vi "Waveform and Laser Controls V7.vi"() -> ()   [LabVIEW 2014]
uses:
  Waveform Scan Parameters.ctl
  <vilib>/Platform/TimedLoop/XDataNode/timing_clust.ctl
  <vilib>/Platform/TimedLoop/XDataNode/nitl_modes.ctl
  <vilib>/Platform/TimedLoop/XDataNode/wakeup.ctl
  <vilib>/rvi/Emulation/niFpgaGetClockAttributes.vi
  <vilib>/rvi/Emulation/niFpgaSctlEmulationGetInTimedLoop.vi
  <vilib>/rvi/Emulation/niFpgaEmulationReportErrorSimple.vi
  <vilib>/rvi/Emulation/niFpgaProcessEmulError.vi
  <vilib>/rvi/eio/common/nirviEmuTemplateMethod_errors.vi
  <vilib>/rvi/Emulation/niFpgaCriticalErrorInLSC.vi
  <vilib>/rvi/Memory/Memory_Emulation/nirvimemoryFastEmulation.vi
  <vilib>/rvi/Memory/Memory_Emulation/nirvimemoryEmulation.vi
  <vilib>/rvi/Emulation/niFpgaEmulationIsFPGAContextNoSignature.vi
  <vilib>/rvi/DataTransferAndStorage/Container/Common/niFpgaContainerGetUniqueNameForEmu.vi
  <vilib>/rvi/errors/nirviReportUnexpectedCaseInternalError (U32).vi
  <vilib>/rvi/Memory/Memory_Emulation/niFpgaMemoryEmulationCacheClearOnFirstRun.vi
  <vilib>/rvi/Memory/Memory_Emulation/nirvimemoryEmulationManagerCache_MakeExclusive.vi
  <vilib>/rvi/Memory/Memory_Emulation/niFpgaMemoryEmulationValidateCache.vi
  <vilib>/rvi/Memory/Memory_Emulation/nirvimemoryEmulationManagerCache_InsertValue.vi
  <vilib>/Utility/error.llb/Clear Errors.vi
  <vilib>/rvi/Memory/Memory_Emulation/nirvimemoryEmulationManagerCache_ReleaseExclusive.vi
  <vilib>/rvi/Memory/Memory_Emulation/nirvimemoryEmulationManagerCache_GetValue.vi
  <vilib>/rvi/Memory/Memory_Emulation/nirvimemoryEmulationManagerCache_SetValue.vi
  <vilib>/eio/EIONode/EIONode.xnode
  <vilib>/rvi/DataTransferAndStorage/Container/XNode/niFpgaContainer.xnode
  <vilib>/Platform/TimedLoop/XDataNode/XDataNode.xnode
  <vilib>/rvi/DataTransferAndStorage/Register/Emulation/niFpgaRegisterEmulation.vi
  <vilib>/Platform/TimedLoop/XDataNode/XDNodeRunTimeDep.lvlib
panel:
  out "frame counter":u16
  in  "Current Frame":u16
  in  "Lower Shutter Command":bool
  in  "Upper Shutter Command":bool
  out "Lower Shutter Status":bool
  out "Upper Shutter Status":bool
  in  "stop":bool
  in  "775 AOM (I16)":i16=16500
  out "Laser Blank Trigger":bool
  in  "Laser On Time (Ticks)":u8=8
  in  "Sequences":u8=4
  in  "Laser Delay (Ticks)":u8
  in  "Laser States":u32
  in  "Blanking Off/Manual":bool
  in  "Z Piezo Axis":i16
  in  "Y Piezo Axis":i16
  in  "X Piezo Axis":i16
  out "End Linear Ramp":bool
  in  "End of Linear Ramp":u32
  in  "Z Stack Start Position (I16)":i16
  in  "Frames Per Z Step":u16
  in  "Number of Z Steps":u16
  in  "Z Step Size (I16)":i16
  in  "Stop Sync Signal":bool
  in  "Accums Per Line":u32[](array[numeric])=[0, 0, 0, 0]
  in  "Number of Lines":u32
  out "Frame Trigger":bool
  in  "Reset Position Error":bool
  in  "Galvo 1 Position (I16)":i16
  in  "Galvo 2 Position (I16)":i16
  in  "WF 3 Data Loaded":bool
  in  "WF 2 Data Loaded":bool
  in  "Waveform Scan Parameters":T1={"Scanning Mode"=0, "Fast Axis WF Length (Elements)"=0, "Fast Axis Sample Period (Ticks)"=40, "Slow Axis 1 WF Length (Elements)"=0, "Slow Axis 1 Sample Period (Ticks)"=40, "Slow Axis 1 Delay (25 ns) Steps"=40, "Slow Axis 2 WFLength (Elements)"=0, "Slow Axis 2 Sample Period (Ticks)"=40, "Slow Axis 2 Delay (25 ns) Steps"=40}
  in  "Resonant Mirror":T2
  in  "Galvo Mirror 2":T3
  in  "Galvo Mirror 1":T3
  in  "Start Waveforms":bool
  in  "Unused Axis Offset":i16
  in  "Slow Axis 2 Waveform Element":i16
  in  "Fast Axis Waveform Element":i16
  in  "Slow Axis 1 Waveform Element":i16
  in  "WF 1 Data Loaded":bool
  # "V2 - Adding in a line clock\nV3 - Cluster Scan Parameters"
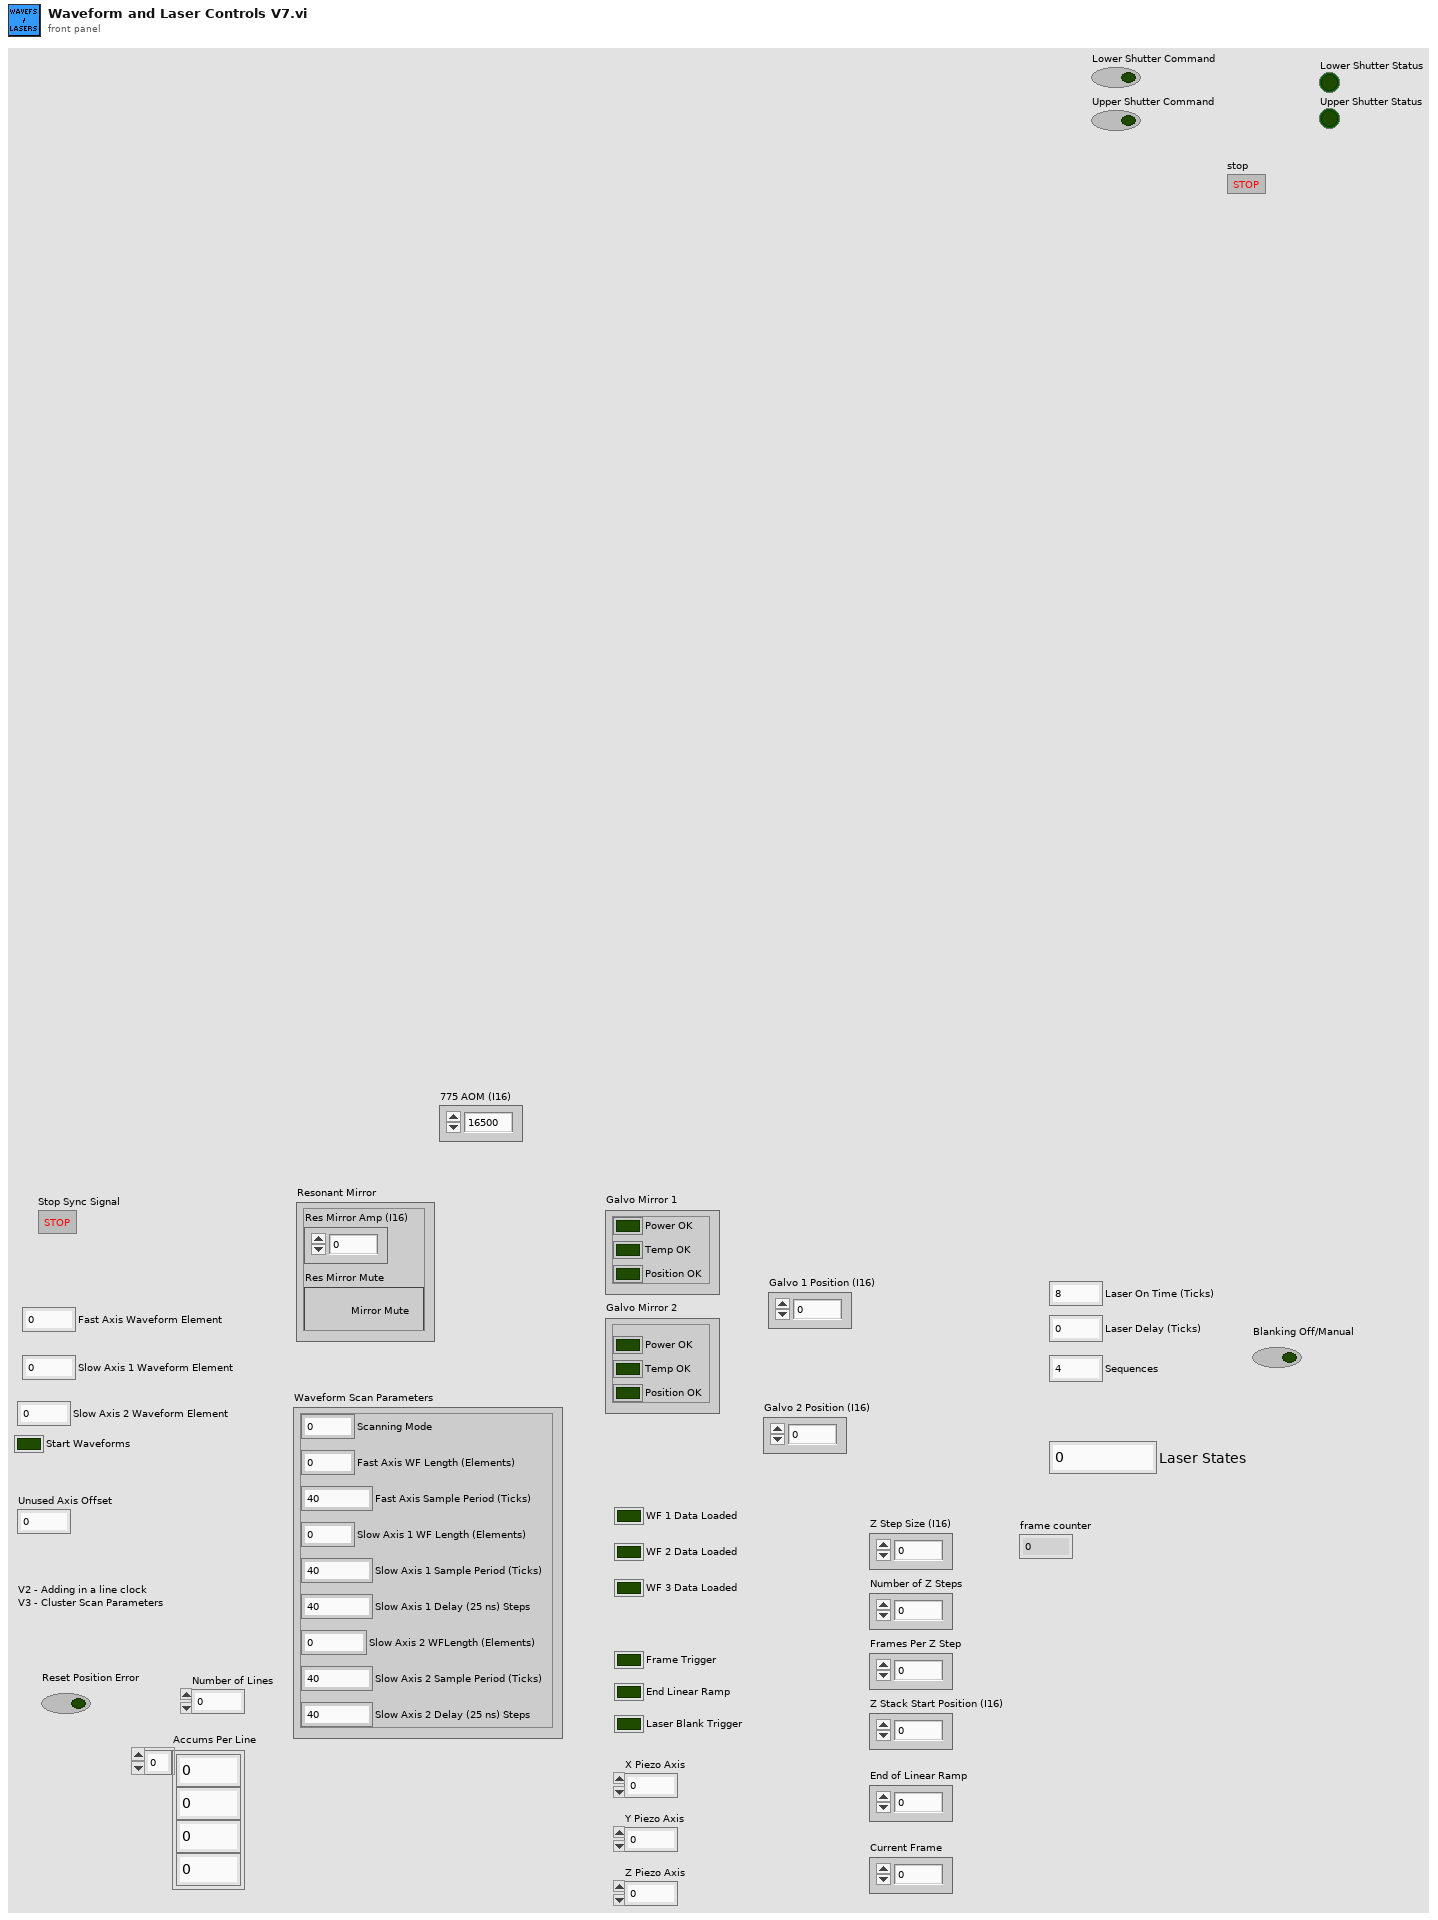
[diagram p1: front panel]
types:
  T1 = typedef "Waveform Scan Parameters.ctl" = cluster{"Scanning Mode":u8, "Fast Axis WF Length (Elements)":i32, "Fast Axis Sample Period (Ticks)":u32, "Slow Axis 1 WF Length (Elements)":i32, "Slow Axis 1 Sample Period (Ticks)":u32, "Slow Axis 1 Delay (25 ns) Steps":i32, "Slow Axis 2 WFLength (Elements)":i32, "Slow Axis 2 Sample Period (Ticks)":u32, "Slow Axis 2 Delay (25 ns) Steps":i32}
  T2 = cluster{"Res Mirror Amp (I16)":i16, "Res Mirror Mute":bool}
  T3 = cluster{"Power OK":bool, "Temp OK":bool, "Position OK":bool}
  T4 = typedef "XDNodeRunTimeDep.lvlib/timing_clust.ctl" = cluster{"Expected End [f-1]":u64, "Actual End [f-1]":u64, "Finished Late? [f-1]":bool, "Expected End [i-1]":u64, "Actual End [i-1]":u64, "Finished Late? [i-1]":bool, "Expected Start [i]":u64, "Actual Start [i]":u64, "Expected Start [f]":u64, "Actual Start [f]":u64, "Source Name":string, "Structure Name":string, "Period":i64, "Deadline":i64, "Offset":i64, "Start":i64, "Priority":i32, "Timeout":i32, "Mode":T5, "Wakeup Reason":T6, "Error":errorcluster, "Source Type":string, "Secondary Source Type":string, "Global End Time":u64, "Global Start Time":u64, "Frame Duration":u64, "Iteration Duration":u64, "Assigned CPU":i32, "I/O Scan Engine Mode":u32}
  T5 = typedef "XDNodeRunTimeDep.lvlib/nitl_modes.ctl" = enum32{"No Change", "Process missed periods, maintain original phase", "Discard missed periods, maintain original phase", "Process missed periods, ignore original phase", "Discard missed periods, ignore original phase"}
  T6 = typedef "XDNodeRunTimeDep.lvlib/wakeup.ctl" = enum32{"Normal", "Aborted", "Asynchronous wakeup", "Timing source error", "Timed loop error", "Timeout"}
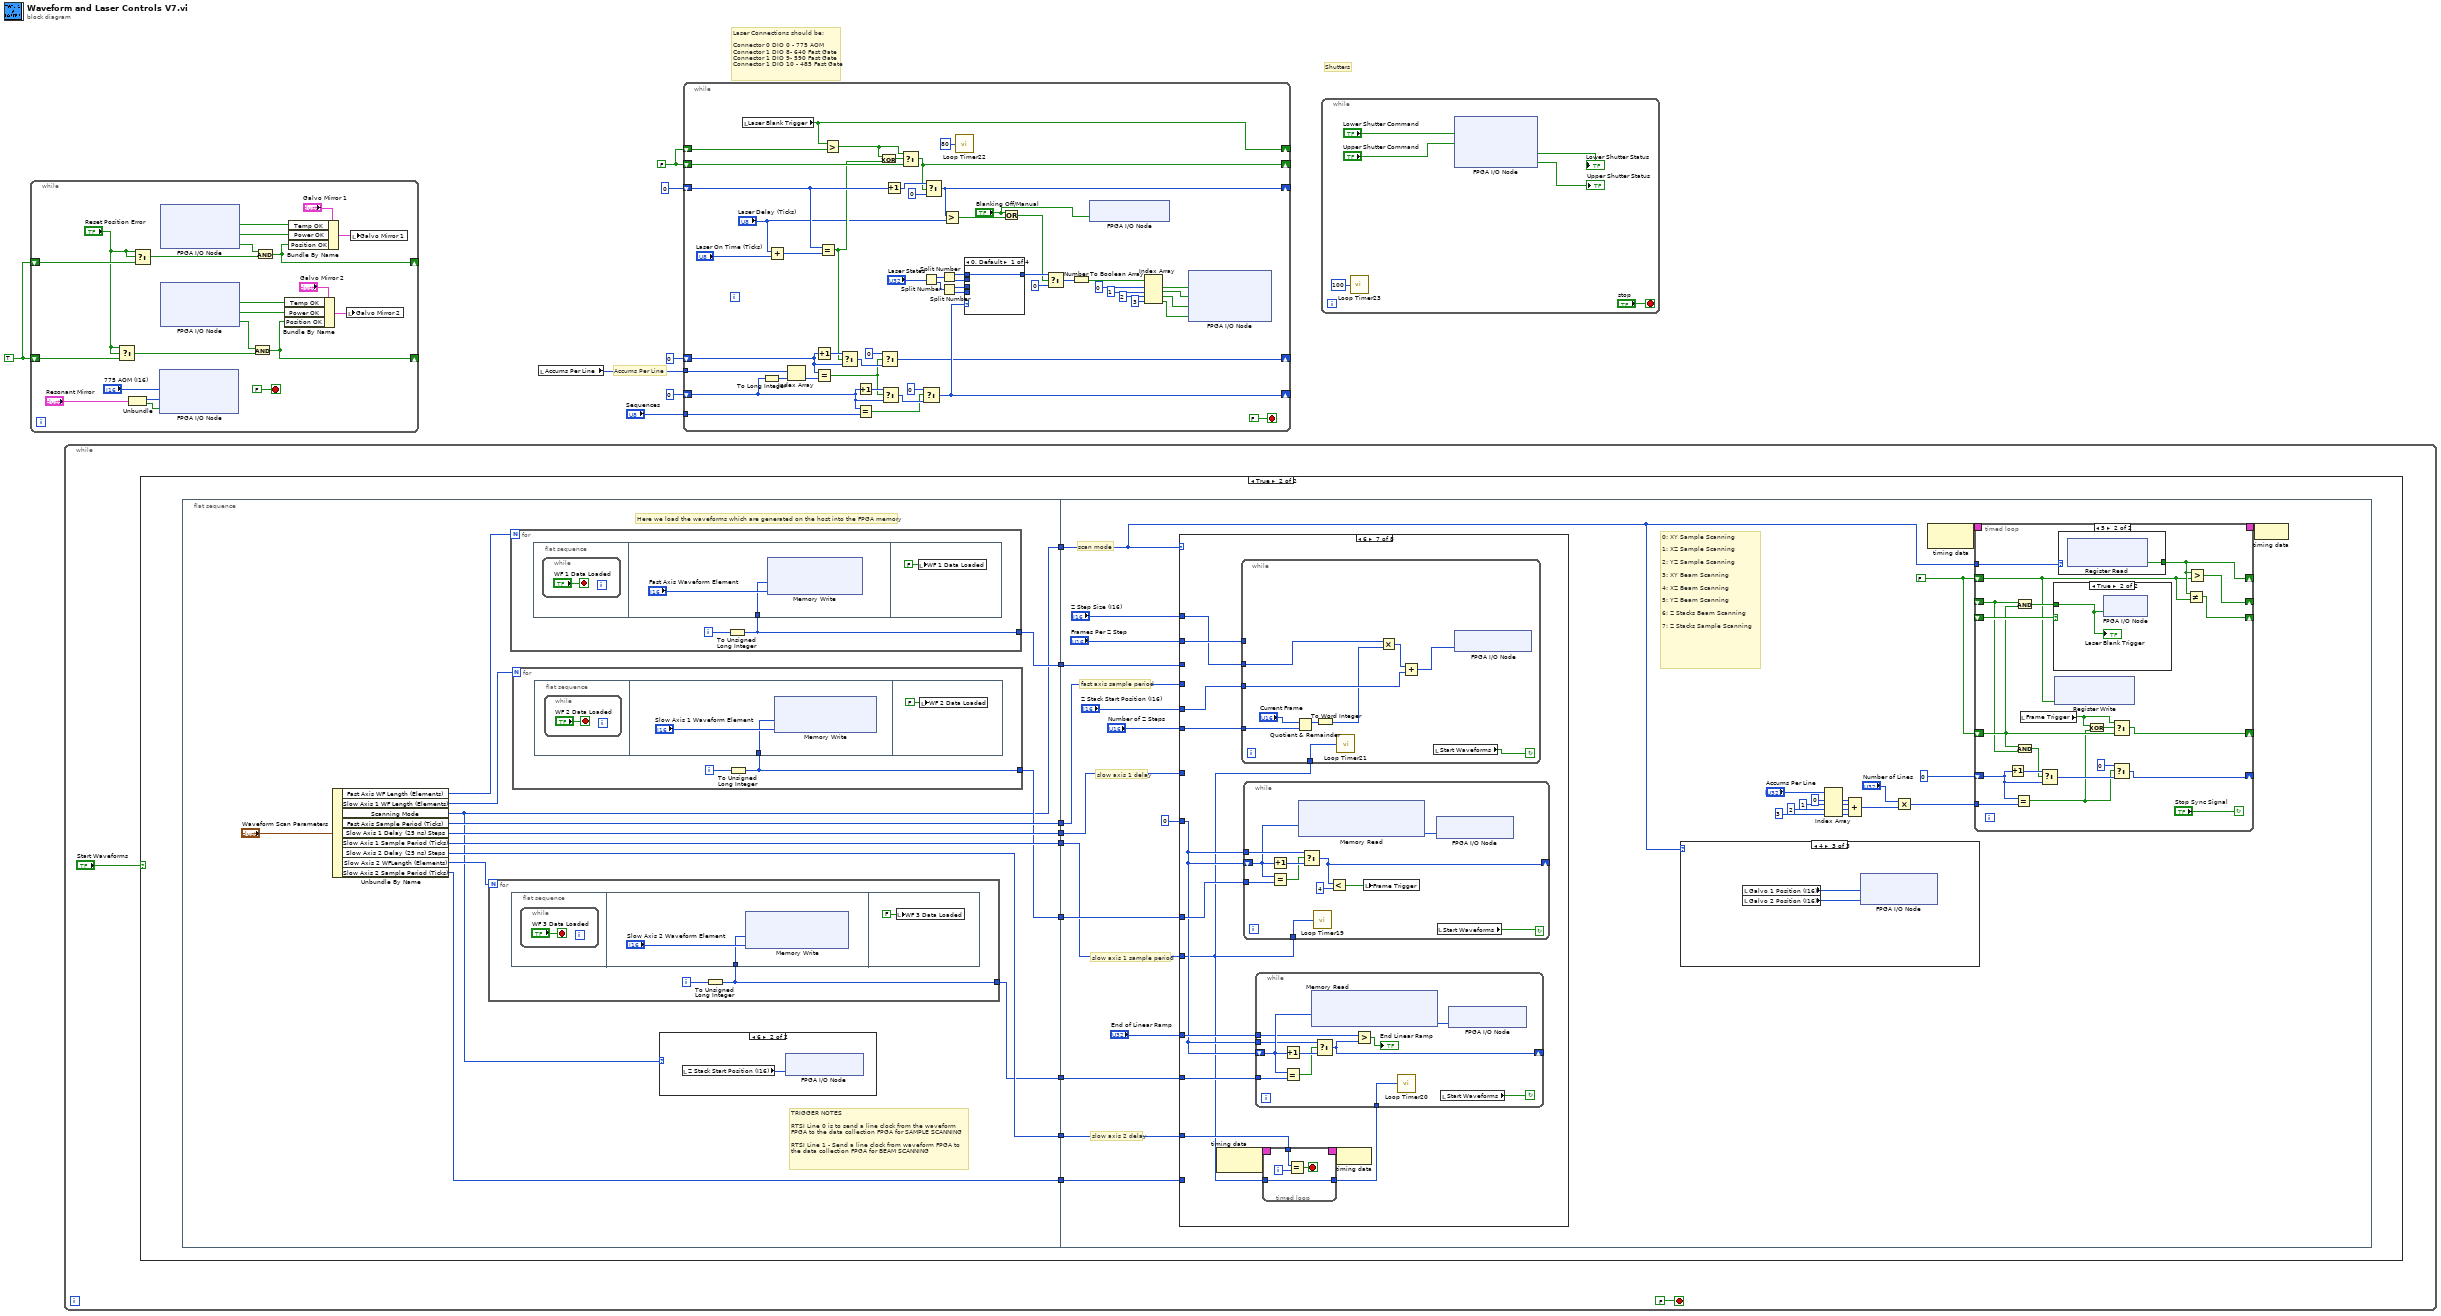
[diagram p0: block diagram]
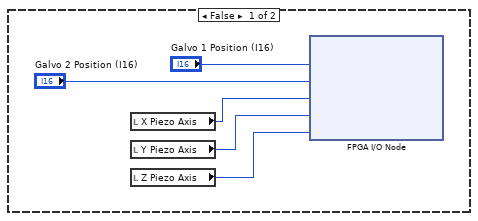
[diagram p5: hidden frame]
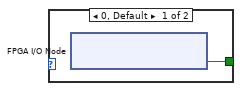
[diagram p7: hidden frame]
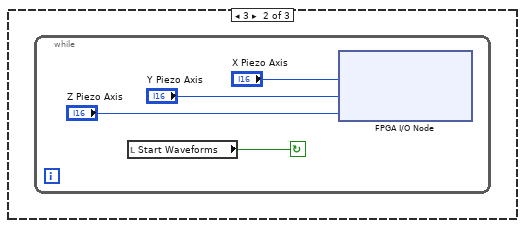
[diagram p10: hidden frame]
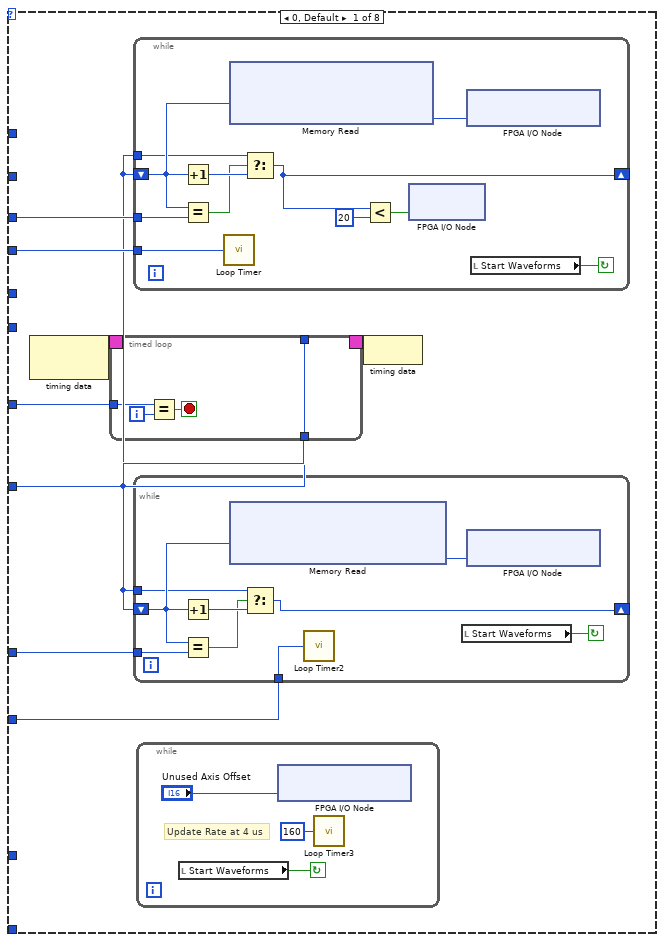
[diagram p11: hidden frame]
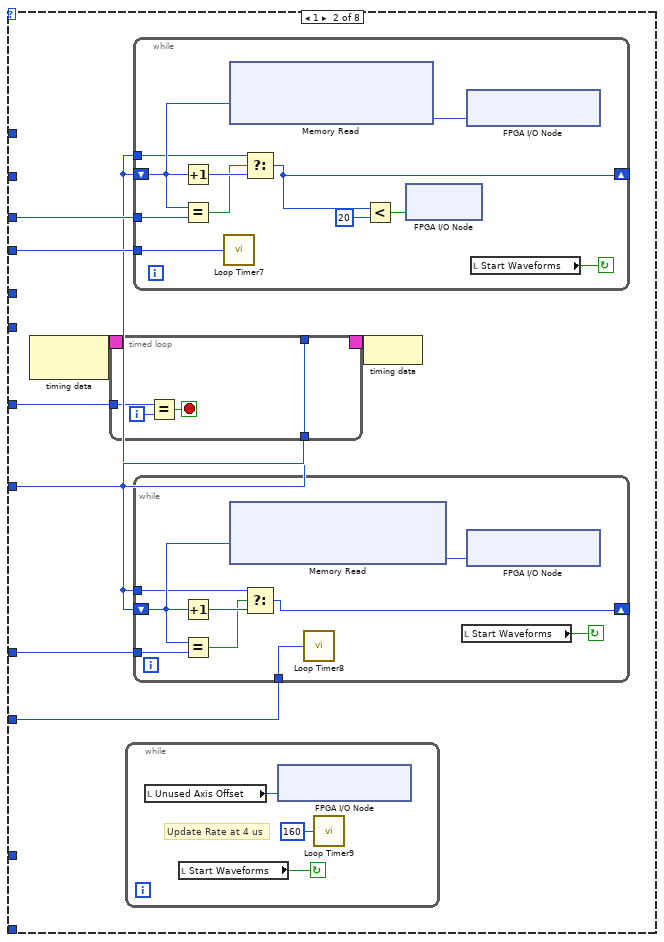
[diagram p12: hidden frame]
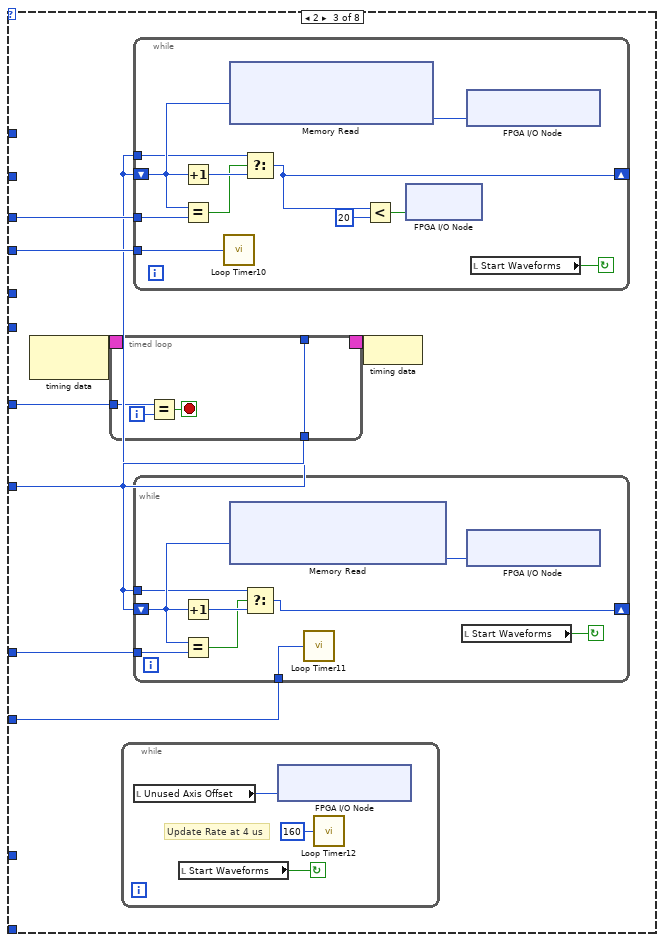
[diagram p13: hidden frame]
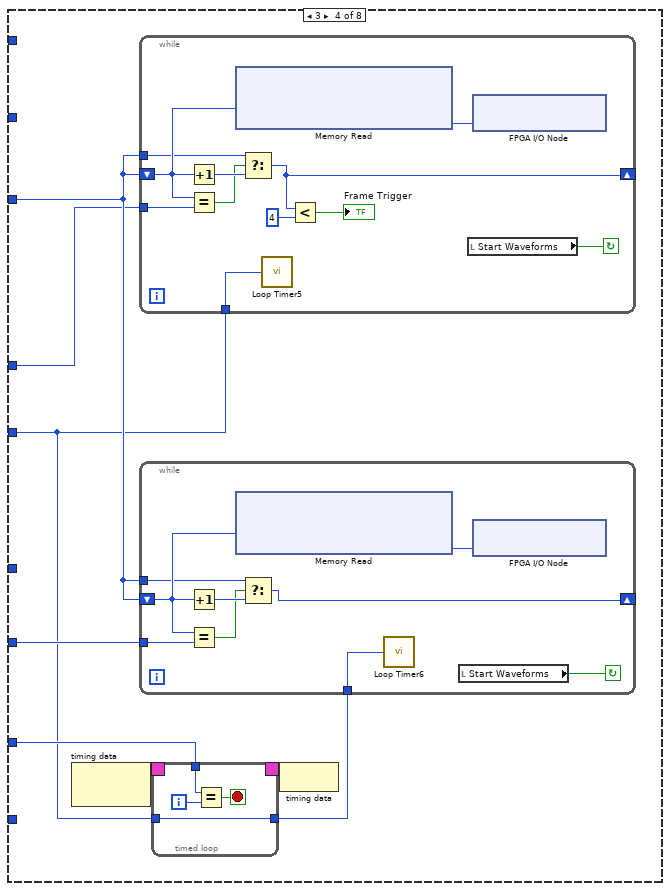
[diagram p14: hidden frame]
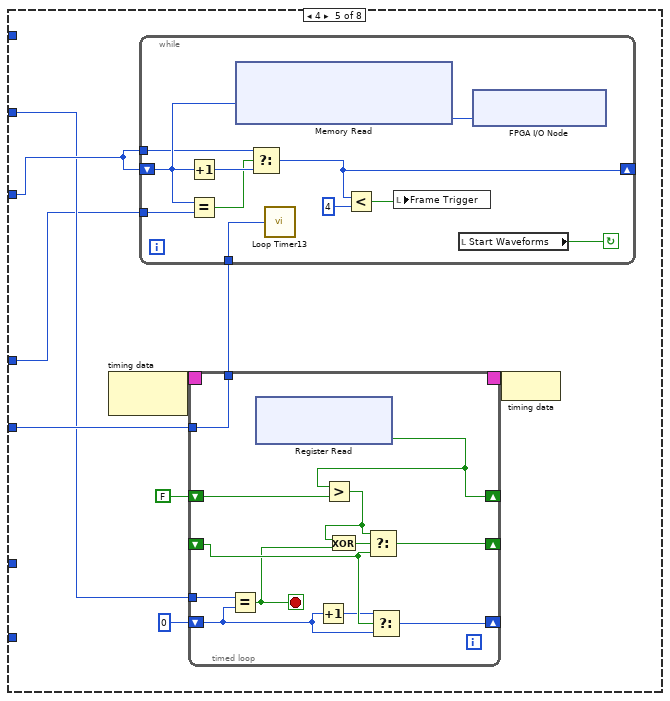
[diagram p15: hidden frame]
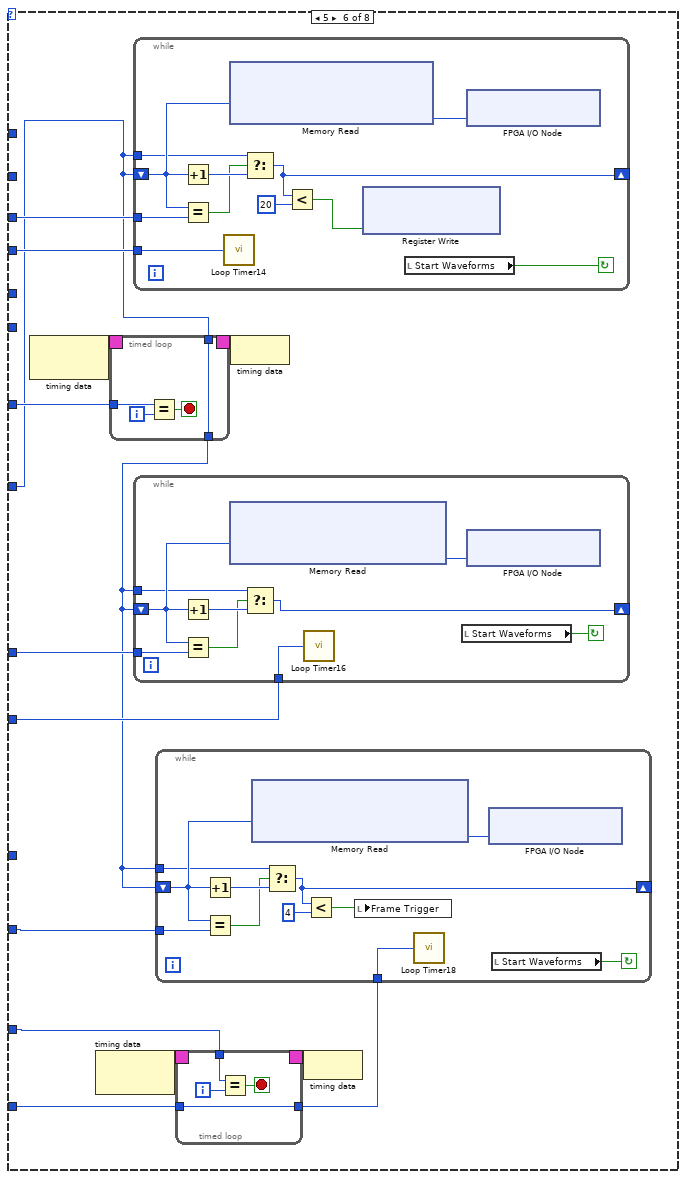
[diagram p16: hidden frame]
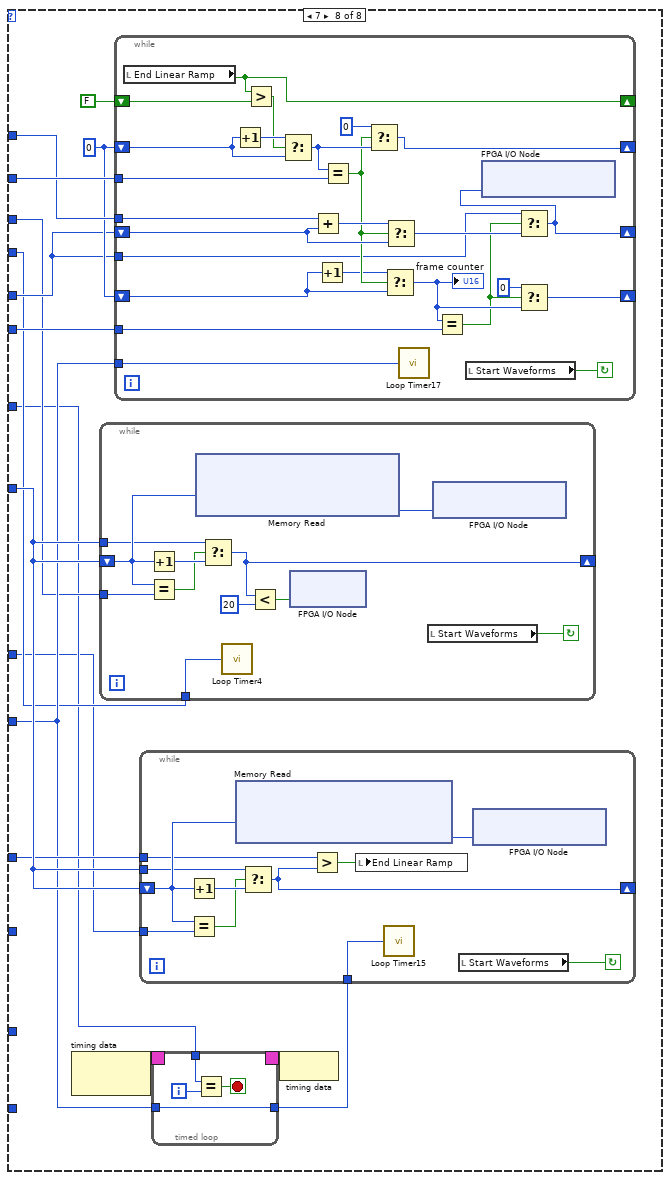
[diagram p17: hidden frame]
diagram:
  w2 = FALSE
  w7 = TRUE
  # "Shutters"
  # "Laser Connections should be:\n\nConnector 0 DIO 0 - 775 AOM\nConnector 1 DIO 8- 640 Fast Gate\nConnector 1 DIO 9- 590 Fast Gate\nConnector 1 DIO 10 - 485 Fast Gate"
  # "Accums Per Line"
  n1 = while {
    shift-right: [w15] -> _
    shift-left: w7 -> [w17]
    shift-right: [w11] -> _
    shift-left: w7 -> [w13]
    stop <- FALSE stop-if-true
    n2 = Select(t="Reset Position Error", s="Reset Position Error", f=w17) -> (s? t:f=w16:bool)
    n3 = Unbundle("Resonant Mirror") -> ("Res Mirror Amp (I16)"=w27:i16, "Res Mirror Mute"=w26:bool)
    n4 = Select(t="Reset Position Error", s="Reset Position Error", f=w13) -> (s? t:f=w12:bool)
    n5 = xnode "FPGA I/O Node"("Connector0/AO4"="775 AOM (I16)", "Connector0/AO7"=w27, "Connector0/DIO7"=w26) -> ()  [unwired: 4 in, 4 out]
    n6 = xnode "FPGA I/O Node"() -> ("Connector0/DIO1"=w8:bool, "Connector0/DIO2"=w25:bool, "Connector0/DIO3"=w14:bool)  [unwired: 4 in, 4 out]
    n7 = xnode "FPGA I/O Node"() -> ("Connector0/DIO4"=w19:bool, "Connector0/DIO5"=w20:bool, "Connector0/DIO6"=w18:bool)  [unwired: 4 in, 4 out]
    n8 = And(x=w18, y=w16) -> (x .and. y?=w15:bool)
    n9 = And(x=w14, y=w12) -> (x .and. y?=w11:bool)
    n10 = Bundle By Name(cluster="Galvo Mirror 2", "Temp OK"=w19, "Power OK"=w20, "Position OK"=w15) -> (w22:T3)
    n11 = Bundle By Name(cluster="Galvo Mirror 1", "Temp OK"=w8, "Power OK"=w25, "Position OK"=w11) -> (w24:T3)
    n12 = local write "Galvo Mirror 2"(w22) -> ()
    n13 = local write "Galvo Mirror 1"(w24) -> ()
  }
  n14 = while {
    stop <- FALSE stop-if-true
    n15 = case shown="True" "Start Waveforms" {
      frame False {
        n16 = local read "X Piezo Axis"() -> (w34:i16)
        n17 = local read "Y Piezo Axis"() -> (w33:i16)
        n18 = local read "Z Piezo Axis"() -> (w32:i16)
        n19 = xnode "FPGA I/O Node"("Connector0/AO5"="Galvo 1 Position (I16)", "Connector0/AO6"="Galvo 2 Position (I16)", "Connector0/AO1"=w34, "Connector0/AO2"=w33, "Connector0/AO3"=w32) -> ()  [unwired: 5 in, 5 out]
      }
      frame True {
        n20 = flat-sequence {
          tunnel: [w58] -> w45
          tunnel: [w48] -> w44
          tunnel: [w49] -> w43
          tunnel: [w47] -> w42
          tunnel: [w56] -> w41
          tunnel: [w55] -> w40
          tunnel: [w54] -> w39
          tunnel: [w53] -> w38
          tunnel: [w46] -> w37
          tunnel: w45 -> [w108]
          tunnel: w44 -> [w107]
          tunnel: w43 -> [w105]
          tunnel: w42 -> [w79]
          tunnel: w41 -> [w104]
          tunnel: w40 -> [w103]
          tunnel: w39 -> [w102]
          tunnel: w38 -> [w101]
          tunnel: w37 -> [w78]
          frame #0 {
            # "TRIGGER NOTES\n\nRTSI Line 0 is to send a line clock from the waveform\nFPGA to the data collection FPGA for SAMPLE SCANNING\n\nRTSI Line 1 - Send a line clock from waveform FPGA to\nthe data collection FPGA for BEAM SCANNING"
            # "Here we load the waveforms which are generated on the host into the FPGA memory"
            n21 = Unbundle By Name("Waveform Scan Parameters") -> ("Fast Axis WF Length (Elements)"=w52:i32, "Slow Axis 1 WF Length (Elements)"=w51:i32, "Scanning Mode"=w47:u8, "Fast Axis Sample Period (Ticks)"=w56:u32, "Slow Axis 1 Delay (25 ns) Steps"=w55:i32, "Slow Axis 1 Sample Period (Ticks)"=w54:u32, "Slow Axis 2 Delay (25 ns) Steps"=w53:i32, "Slow Axis 2 WFLength (Elements)"=w50:i32, "Slow Axis 2 Sample Period (Ticks)"=w46:u32)
            n22 = for {
              N: w50 -> [_]
              tunnel: [w60] -> w48
              i -> [w61]
              n23 = flat-sequence {
                tunnel: w60 -> [w63]
                frame #0 {
                  n24 = while {
                    stop <- "WF 3 Data Loaded" stop-if-true
                  }
                }
                frame #1 {
                  n25 = xnode ("Memory Write")("Address"=w63, "Data"="Slow Axis 2 Waveform Element") -> ()  [unwired: 1 in, 1 out]
                }
                frame #2 {
                  n26 = local write "WF 3 Data Loaded"(FALSE ("Host Data Loaded")) -> ()
                }
              }
              n27 = To Unsigned Long Integer(number=w61) -> (unsigned 32bit integer=w60:u32)
            }
            n28 = for {
              N: w52 -> [_]
              tunnel: [w72] -> w58
              i -> [w73]
              n29 = flat-sequence {
                tunnel: w72 -> [w75]
                frame #0 {
                  n30 = while {
                    stop <- "WF 1 Data Loaded" stop-if-true
                  }
                }
                frame #1 {
                  n31 = xnode ("Memory Write")("Address"=w75, "Data"="Fast Axis Waveform Element") -> ()  [unwired: 1 in, 1 out]
                }
                frame #2 {
                  n32 = local write "WF 1 Data Loaded"(FALSE ("Host Data Loaded")) -> ()
                }
              }
              n33 = To Unsigned Long Integer(number=w73) -> (unsigned 32bit integer=w72:u32)
            }
            n34 = for {
              N: w51 -> [_]
              tunnel: [w66] -> w49
              i -> [w67]
              n35 = flat-sequence {
                tunnel: w66 -> [w69]
                frame #0 {
                  n36 = while {
                    stop <- "WF 2 Data Loaded" stop-if-true
                  }
                }
                frame #1 {
                  n37 = xnode ("Memory Write")("Address"=w69, "Data"="Slow Axis 1 Waveform Element") -> ()  [unwired: 1 in, 1 out]
                }
                frame #2 {
                  n38 = local write "WF 2 Data Loaded"(FALSE ("Host Data Loaded")) -> ()
                }
              }
              n39 = To Unsigned Long Integer(number=w67) -> (unsigned 32bit integer=w66:u32)
            }
            n40 = case shown="6" w47 {
              frame 0, Default {
              }
              frame 6 {
                n41 = local read "Z Stack Start Position (I16)"() -> (w59:i16)
                n42 = xnode "FPGA I/O Node"("Connector0/AO3"=w59) -> ()  [unwired: 1 in, 1 out]
              }
            }
          }
          frame #1 {
            w81 = FALSE
            # "slow axis 2 delay"
            # "slow axis 1 sample period"
            # "slow axis 1 delay"
            # "fast axis sample period"
            # "scan mode"
            # "0: XY Sample Scanning\n\n1: XZ Sample Scanning\n\n2: YZ Sample Scanning\n\n3: XY Beam Scanning\n\n4: XZ Beam Scanning\n\n5: YZ Beam Scanning\n\n6: Z Stacks Beam Scanning\n\n7: Z Stacks Sample Scanning"
            n43 = case shown="6" w79 {
              tunnel: w108 -> [w149 w189 w229 _ _ w349 _ w452]
              tunnel: w104 -> [w148 w188 w228 _ _ w348 _ w453]
              tunnel: w107 -> [_ _ _ w270 _ w343 w409 _]
              tunnel: u32 0 -> [w143 w183 w223 w269 w307 w345 w399 w465]
              tunnel: w103 -> [w147 w187 w227 _ w305 w347 _ w451]
              tunnel: w101 -> [_ _ _ w268 _ w342 w408 _]
              tunnel: w105 -> [w145 w185 w225 w263 w304 w346 w405 w450]
              tunnel: w102 -> [w144 w184 w224 w264 w306 w344 w397 w454]
              tunnel: "Frames Per Z Step" -> [_ _ _ _ _ _ w404 w461]
              tunnel: "Z Stack Start Position (I16)" -> [_ _ _ _ _ _ w400 w457]
              tunnel: "Z Step Size (I16)" -> [_ _ _ _ _ _ w403 w460]
              tunnel: "Number of Z Steps" -> [_ _ _ _ _ _ w402 w458]
              tunnel: "End of Linear Ramp" -> [_ _ _ _ _ _ w401 w456]
              tunnel: w78 -> [_ _ _ _ _ w335 _ _]
              frame 0, Default {
                n44 = node-c288() -> (w151:T4)  [unwired: 1 in]
                n45 = timed-loop {
                  timing: w151 -> [_]
                  timing-out: [_] -> w150
                  tunnel: w147 -> [w156]
                  tunnel: w143 -> [w155]
                  tunnel: [w155] -> w146
                  i -> [w158]
                  stop <- w157 stop-if-true
                  n46 = Equal?(x=w156, y=w158) -> (x = y?=w157:bool)
                }
                n47 = while {
                  shift-right: [w174] -> _
                  shift-left: w143 -> [w180]
                  tunnel: w149 -> [w181]
                  tunnel: w148 -> [w178]
                  tunnel: w143 -> [w177]
                  stop <- w176 continue-if-true
                  n48 = Increment(x=w180) -> (x+1=w182:u32)
                  n49 = Equal?(x=w180, y=w181) -> (x = y?=w175:bool)
                  n50 = call "Loop Timer"("Count(Ticks)"=w178) -> ()  [unwired: 1 out]
                  n51 = xnode ("Memory Read")("Address"=w180) -> ("Data"=w179:i16)  [unwired: 1 in, 1 out]
                  n52 = Select(t=w177, s=w175, f=w182) -> (s? t:f=w174:u32)
                  n53 = Less?(x=w174, y=u32 20) -> (x < y?=w172:bool)
                  n54 = xnode "FPGA I/O Node"("TRIG0"=w172) -> ()  [unwired: 1 in, 1 out]
                  n55 = xnode "FPGA I/O Node"("Connector0/AO1"=w179) -> ()  [unwired: 1 in, 1 out]
                  n56 = local read "Start Waveforms"() -> (w176:bool)
                }
                n57 = while {
                  shift-right: [w170] -> _
                  shift-left: w146 -> [w167]
                  tunnel: w145 -> [w169]
                  tunnel: w146 -> [w165]
                  tunnel: w144 -> [w164]
                  stop <- w163 continue-if-true
                  n58 = Increment(x=w167) -> (x+1=w171:u32)
                  n59 = Equal?(x=w167, y=w169) -> (x = y?=w168:bool)
                  n60 = xnode ("Memory Read")("Address"=w167) -> ("Data"=w166:i16)  [unwired: 1 in, 1 out]
                  n61 = Select(t=w165, s=w168, f=w171) -> (s? t:f=w170:u32)
                  n62 = call "Loop Timer2"("Count(Ticks)"=w164) -> ()  [unwired: 1 out]
                  n63 = local read "Start Waveforms"() -> (w163:bool)
                  n64 = xnode "FPGA I/O Node"("Connector0/AO2"=w166) -> ()  [unwired: 1 in, 1 out]
                }
                n65 = while {
                  stop <- w152 continue-if-true
                  # "Update Rate at 4 us"
                  n66 = local read "Start Waveforms"() -> (w152:bool)
                  n67 = xnode "FPGA I/O Node"("Connector0/AO3"="Unused Axis Offset") -> ()  [unwired: 1 in, 1 out]
                  n68 = call "Loop Timer3"("Count(Ticks)"=u32 160) -> ()  [unwired: 1 out]
                }
                n69 = node-c288(w150) -> ()
              }
              frame 1 {
                n70 = node-c288() -> (w191:T4)  [unwired: 1 in]
                n71 = timed-loop {
                  timing: w191 -> [_]
                  timing-out: [_] -> w190
                  tunnel: w187 -> [w196]
                  tunnel: w183 -> [w195]
                  tunnel: [w195] -> w186
                  i -> [w198]
                  stop <- w197 stop-if-true
                  n72 = Equal?(x=w196, y=w198) -> (x = y?=w197:bool)
                }
                n73 = while {
                  stop <- w193 continue-if-true
                  # "Update Rate at 4 us"
                  n74 = local read "Unused Axis Offset"() -> (w192:i16)
                  n75 = local read "Start Waveforms"() -> (w193:bool)
                  n76 = xnode "FPGA I/O Node"("Connector0/AO2"=w192) -> ()  [unwired: 1 in, 1 out]
                  n77 = call "Loop Timer9"("Count(Ticks)"=u32 160) -> ()  [unwired: 1 out]
                }
                n78 = while {
                  shift-right: [w214] -> _
                  shift-left: w183 -> [w220]
                  tunnel: w189 -> [w221]
                  tunnel: w188 -> [w218]
                  tunnel: w183 -> [w217]
                  stop <- w216 continue-if-true
                  n79 = Increment(x=w220) -> (x+1=w222:u32)
                  n80 = Equal?(x=w220, y=w221) -> (x = y?=w215:bool)
                  n81 = call "Loop Timer7"("Count(Ticks)"=w218) -> ()  [unwired: 1 out]
                  n82 = xnode ("Memory Read")("Address"=w220) -> ("Data"=w219:i16)  [unwired: 1 in, 1 out]
                  n83 = Select(t=w217, s=w215, f=w222) -> (s? t:f=w214:u32)
                  n84 = Less?(x=w214, y=u32 20) -> (x < y?=w212:bool)
                  n85 = xnode "FPGA I/O Node"("TRIG0"=w212) -> ()  [unwired: 1 in, 1 out]
                  n86 = xnode "FPGA I/O Node"("Connector0/AO1"=w219) -> ()  [unwired: 1 in, 1 out]
                  n87 = local read "Start Waveforms"() -> (w216:bool)
                }
                n88 = while {
                  shift-right: [w210] -> _
                  shift-left: w186 -> [w207]
                  tunnel: w185 -> [w209]
                  tunnel: w186 -> [w205]
                  tunnel: w184 -> [w204]
                  stop <- w203 continue-if-true
                  n89 = Increment(x=w207) -> (x+1=w211:u32)
                  n90 = Equal?(x=w207, y=w209) -> (x = y?=w208:bool)
                  n91 = xnode ("Memory Read")("Address"=w207) -> ("Data"=w206:i16)  [unwired: 1 in, 1 out]
                  n92 = Select(t=w205, s=w208, f=w211) -> (s? t:f=w210:u32)
                  n93 = call "Loop Timer8"("Count(Ticks)"=w204) -> ()  [unwired: 1 out]
                  n94 = local read "Start Waveforms"() -> (w203:bool)
                  n95 = xnode "FPGA I/O Node"("Connector0/AO3"=w206) -> ()  [unwired: 1 in, 1 out]
                }
                n96 = node-c288(w190) -> ()
              }
              frame 2 {
                n97 = node-c288() -> (w231:T4)  [unwired: 1 in]
                n98 = timed-loop {
                  timing: w231 -> [_]
                  timing-out: [_] -> w230
                  tunnel: w227 -> [w236]
                  tunnel: w223 -> [w235]
                  tunnel: [w235] -> w226
                  i -> [w238]
                  stop <- w237 stop-if-true
                  n99 = Equal?(x=w236, y=w238) -> (x = y?=w237:bool)
                }
                n100 = while {
                  stop <- w233 continue-if-true
                  # "Update Rate at 4 us"
                  n101 = local read "Unused Axis Offset"() -> (w232:i16)
                  n102 = local read "Start Waveforms"() -> (w233:bool)
                  n103 = xnode "FPGA I/O Node"("Connector0/AO1"=w232) -> ()  [unwired: 1 in, 1 out]
                  n104 = call "Loop Timer12"("Count(Ticks)"=u32 160) -> ()  [unwired: 1 out]
                }
                n105 = while {
                  shift-right: [w254] -> _
                  shift-left: w223 -> [w260]
                  tunnel: w229 -> [w261]
                  tunnel: w228 -> [w258]
                  tunnel: w223 -> [w257]
                  stop <- w256 continue-if-true
                  n106 = Increment(x=w260) -> (x+1=w262:u32)
                  n107 = Equal?(x=w260, y=w261) -> (x = y?=w255:bool)
                  n108 = call "Loop Timer10"("Count(Ticks)"=w258) -> ()  [unwired: 1 out]
                  n109 = xnode ("Memory Read")("Address"=w260) -> ("Data"=w259:i16)  [unwired: 1 in, 1 out]
                  n110 = Select(t=w257, s=w255, f=w262) -> (s? t:f=w254:u32)
                  n111 = Less?(x=w254, y=u32 20) -> (x < y?=w252:bool)
                  n112 = xnode "FPGA I/O Node"("TRIG0"=w252) -> ()  [unwired: 1 in, 1 out]
                  n113 = xnode "FPGA I/O Node"("Connector0/AO2"=w259) -> ()  [unwired: 1 in, 1 out]
                  n114 = local read "Start Waveforms"() -> (w256:bool)
                }
                n115 = while {
                  shift-right: [w250] -> _
                  shift-left: w226 -> [w247]
                  tunnel: w225 -> [w249]
                  tunnel: w226 -> [w245]
                  tunnel: w224 -> [w244]
                  stop <- w243 continue-if-true
                  n116 = Increment(x=w247) -> (x+1=w251:u32)
                  n117 = Equal?(x=w247, y=w249) -> (x = y?=w248:bool)
                  n118 = xnode ("Memory Read")("Address"=w247) -> ("Data"=w246:i16)  [unwired: 1 in, 1 out]
                  n119 = Select(t=w245, s=w248, f=w251) -> (s? t:f=w250:u32)
                  n120 = call "Loop Timer11"("Count(Ticks)"=w244) -> ()  [unwired: 1 out]
                  n121 = local read "Start Waveforms"() -> (w243:bool)
                  n122 = xnode "FPGA I/O Node"("Connector0/AO3"=w246) -> ()  [unwired: 1 in, 1 out]
                }
                n123 = node-c288(w230) -> ()
              }
              frame 3 {
                n124 = node-c288() -> (w267:T4)  [unwired: 1 in]
                n125 = while {
                  shift-right: [w290] -> _
                  shift-left: w269 -> [w296]
                  tunnel: w263 -> [w297]
                  tunnel: w264 -> [w294]
                  tunnel: w269 -> [w293]
                  stop <- w292 continue-if-true
                  n126 = Increment(x=w296) -> (x+1=w298:u32)
                  n127 = Equal?(x=w296, y=w297) -> (x = y?=w291:bool)
                  n128 = xnode ("Memory Read")("Address"=w296) -> ("Data"=w295:i16)  [unwired: 1 in, 1 out]
                  n129 = Select(t=w293, s=w291, f=w298) -> (s? t:f=w290:u32)
                  n130 = call "Loop Timer5"("Count(Ticks)"=w294) -> ()  [unwired: 1 out]
                  n131 = Less?(x=w290, y=u32 4) -> (x < y?=→"Frame Trigger":bool)
                  n132 = local read "Start Waveforms"() -> (w292:bool)
                  n133 = xnode "FPGA I/O Node"("Connector0/AO5"=w295) -> ()  [unwired: 1 in, 1 out]
                }
                n134 = timed-loop {
                  timing: w267 -> [_]
                  timing-out: [_] -> w266
                  tunnel: w264 -> [w280]
                  tunnel: [w280] -> w265
                  tunnel: w268 -> [w281]
                  i -> [w283]
                  stop <- w282 stop-if-true
                  n135 = Equal?(x=w281, y=w283) -> (x = y?=w282:bool)
                }
                n136 = while {
                  shift-right: [w278] -> _
                  shift-left: w269 -> [w276]
                  tunnel: w270 -> [w277]
                  tunnel: w265 -> [w274]
                  tunnel: w269 -> [w273]
                  stop <- w272 continue-if-true
                  n137 = Increment(x=w276) -> (x+1=w279:u32)
                  n138 = Equal?(x=w276, y=w277) -> (x = y?=w271:bool)
                  n139 = xnode ("Memory Read")("Address"=w276) -> ("Data"=w275:i16)  [unwired: 1 in, 1 out]
                  n140 = Select(t=w273, s=w271, f=w279) -> (s? t:f=w278:u32)
                  n141 = call "Loop Timer6"("Count(Ticks)"=w274) -> ()  [unwired: 1 out]
                  n142 = local read "Start Waveforms"() -> (w272:bool)
                  n143 = xnode "FPGA I/O Node"("Connector0/AO6"=w275) -> ()  [unwired: 1 in, 1 out]
                }
                n144 = node-c288(w266) -> ()
              }
              frame 4 {
                n145 = node-c288() -> (w302:T4)  [unwired: 1 in]
                n146 = timed-loop {
                  timing: w302 -> [_]
                  timing-out: [_] -> w301
                  tunnel: w306 -> [w310]
                  shift-right: [w308] -> _
                  shift-left: FALSE -> [w319]
                  shift-right: [w316] -> _
                  shift-left: _ -> [w315]
                  shift-right: [w313] -> _
                  shift-left: 0 -> [w311]
                  tunnel: w305 -> [w312]
                  tunnel: [w310] -> w303
                  stop <- w309 stop-if-true
                  n147 = Equal?(x=w312, y=w311) -> (x = y?=w309:bool)
                  n148 = xnode ("Register Read")() -> ("Data"=w308:bool)  [unwired: 1 in, 1 out]
                  n149 = Increment(x=w311) -> (x+1=w314:i32)
                  n150 = Greater?(x=w308, y=w319) -> (0:w317:bool)
                  n151 = Exclusive Or(1:w309, 2:w317) -> (0:w318:bool)
                  n152 = Select(t=w317, s=w318, f=w315) -> (s? t:f=w316:bool)
                  n153 = Select(t=w314, s=w315, f=w311) -> (s? t:f=w313:i32)
                }
                n154 = while {
                  shift-right: [w325] -> _
                  shift-left: w307 -> [w331]
                  tunnel: w304 -> [w333]
                  tunnel: w303 -> [w329]
                  tunnel: w307 -> [w328]
                  stop <- w327 continue-if-true
                  n155 = Increment(x=w331) -> (x+1=w334:u32)
                  n156 = Equal?(x=w331, y=w333) -> (x = y?=w332:bool)
                  n157 = xnode ("Memory Read")("Address"=w331) -> ("Data"=w330:i16)  [unwired: 1 in, 1 out]
                  n158 = Select(t=w328, s=w332, f=w334) -> (s? t:f=w325:u32)
                  n159 = call "Loop Timer13"("Count(Ticks)"=w329) -> ()  [unwired: 1 out]
                  n160 = Less?(x=w325, y=u32 4) -> (x < y?=w324:bool)
                  n161 = local write "Frame Trigger"(w324) -> ()
                  n162 = local read "Start Waveforms"() -> (w327:bool)
                  n163 = xnode "FPGA I/O Node"("Connector0/AO3"=w330) -> ()  [unwired: 1 in, 1 out]
                }
                n164 = node-c288(w301) -> ()
              }
              frame 5 {
                n165 = node-c288() -> (w341:T4)  [unwired: 1 in]
                n166 = node-c288() -> (w339:T4)  [unwired: 1 in]
                n167 = timed-loop {
                  timing: w341 -> [_]
                  timing-out: [_] -> w340
                  tunnel: w347 -> [w370]
                  tunnel: w345 -> [w369]
                  tunnel: [w369] -> w336
                  i -> [w372]
                  stop <- w371 stop-if-true
                  n168 = Equal?(x=w370, y=w372) -> (x = y?=w371:bool)
                }
                n169 = while {
                  shift-right: [w389] -> _
                  shift-left: w345 -> [w394]
                  tunnel: w349 -> [w395]
                  tunnel: w348 -> [w392]
                  tunnel: w345 -> [w391]
                  stop <- w387 continue-if-true
                  n170 = Increment(x=w394) -> (x+1=w396:u32)
                  n171 = Equal?(x=w394, y=w395) -> (x = y?=w390:bool)
                  n172 = call "Loop Timer14"("Count(Ticks)"=w392) -> ()  [unwired: 1 out]
                  n173 = xnode ("Memory Read")("Address"=w394) -> ("Data"=w393:i16)  [unwired: 1 in, 1 out]
                  n174 = Select(t=w391, s=w390, f=w396) -> (s? t:f=w389:u32)
                  n175 = Less?(x=w389, y=u32 20) -> (x < y?=w386:bool)
                  n176 = xnode ("Register Write")("Data"=w386) -> ()  [unwired: 1 in, 1 out]
                  n177 = local read "Start Waveforms"() -> (w387:bool)
                  n178 = xnode "FPGA I/O Node"("Connector0/AO5"=w393) -> ()  [unwired: 1 in, 1 out]
                }
                n179 = while {
                  shift-right: [w384] -> _
                  shift-left: w336 -> [w381]
                  tunnel: w346 -> [w383]
                  tunnel: w336 -> [w379]
                  tunnel: w344 -> [w378]
                  stop <- w377 continue-if-true
                  n180 = Increment(x=w381) -> (x+1=w385:u32)
                  n181 = Equal?(x=w381, y=w383) -> (x = y?=w382:bool)
                  n182 = xnode ("Memory Read")("Address"=w381) -> ("Data"=w380:i16)  [unwired: 1 in, 1 out]
                  n183 = Select(t=w379, s=w382, f=w385) -> (s? t:f=w384:u32)
                  n184 = call "Loop Timer16"("Count(Ticks)"=w378) -> ()  [unwired: 1 out]
                  n185 = local read "Start Waveforms"() -> (w377:bool)
                  n186 = xnode "FPGA I/O Node"("Connector0/AO6"=w380) -> ()  [unwired: 1 in, 1 out]
                }
                n187 = timed-loop {
                  timing: w339 -> [_]
                  timing-out: [_] -> w338
                  tunnel: w335 -> [w361]
                  tunnel: [w361] -> w337
                  tunnel: w342 -> [w362]
                  i -> [w364]
                  stop <- w363 stop-if-true
                  n188 = Equal?(x=w362, y=w364) -> (x = y?=w363:bool)
                }
                n189 = while {
                  shift-right: [w352] -> _
                  shift-left: w336 -> [w357]
                  tunnel: w343 -> [w359]
                  tunnel: w337 -> [w355]
                  tunnel: w336 -> [w354]
                  stop <- w353 continue-if-true
                  n190 = Increment(x=w357) -> (x+1=w360:u32)
                  n191 = Equal?(x=w357, y=w359) -> (x = y?=w358:bool)
                  n192 = xnode ("Memory Read")("Address"=w357) -> ("Data"=w356:i16)  [unwired: 1 in, 1 out]
                  n193 = Select(t=w354, s=w358, f=w360) -> (s? t:f=w352:u32)
                  n194 = Less?(x=w352, y=u32 4) -> (x < y?=w350:bool)
                  n195 = local write "Frame Trigger"(w350) -> ()
                  n196 = call "Loop Timer18"("Count(Ticks)"=w355) -> ()  [unwired: 1 out]
                  n197 = xnode "FPGA I/O Node"("Connector0/AO3"=w356) -> ()  [unwired: 1 in, 1 out]
                  n198 = local read "Start Waveforms"() -> (w353:bool)
                }
                n199 = node-c288(w340) -> ()
                n200 = node-c288(w338) -> ()
              }
              frame 6 {
                n201 = node-c288() -> (w407:T4)  [unwired: 1 in]
                n202 = while {
                  tunnel: w404 -> [_]
                  tunnel: w403 -> [w423]
                  tunnel: w400 -> [w424]
                  tunnel: w402 -> [w427]
                  tunnel: w397 -> [w429]
                  stop <- w430 continue-if-true
                  n203 = Quotient & Remainder(x="Current Frame", y=w427) -> (x-y*floor(x/y)=w422:u16)  [unwired: 1 out]
                  n204 = To Word Integer(number=w422) -> (16bit integer=w421:i16)
                  n205 = call "Loop Timer21"("Count(Ticks)"=w429) -> ()  [unwired: 1 out]
                  n206 = Multiply(x=w423, y=w421) -> (x*y=w426:i16)
                  n207 = Add(x=w426, y=w424) -> (x+y=w425:i16)
                  n208 = local read "Start Waveforms"() -> (w430:bool)
                  n209 = xnode "FPGA I/O Node"("Connector0/AO3"=w425) -> ()  [unwired: 1 in, 1 out]
                }
                n210 = while {
                  tunnel: w399 -> [w420]
                  tunnel: w405 -> [w419]
                  tunnel: w397 -> [w418]
                  shift-right: [w416] -> _
                  shift-left: w399 -> [w417]
                  stop <- w410 continue-if-true
                  n211 = Increment(x=w417) -> (x+1=w415:u32)
                  n212 = Equal?(x=w417, y=w419) -> (x = y?=w413:bool)
                  n213 = xnode ("Memory Read")("Address"=w417) -> ("Data"=w414:i16)  [unwired: 1 in, 1 out]
                  n214 = Select(t=w420, s=w413, f=w415) -> (s? t:f=w416:u32)
                  n215 = call "Loop Timer19"("Count(Ticks)"=w418) -> ()  [unwired: 1 out]
                  n216 = Less?(x=w416, y=u32 4) -> (x < y?=w411:bool)
                  n217 = local write "Frame Trigger"(w411) -> ()
                  n218 = xnode "FPGA I/O Node"("Connector0/AO5"=w414) -> ()  [unwired: 1 in, 1 out]
                  n219 = local read "Start Waveforms"() -> (w410:bool)
                }
                n220 = timed-loop {
                  timing: w407 -> [_]
                  timing-out: [_] -> w406
                  tunnel: w397 -> [w442]
                  tunnel: [w442] -> w398
                  tunnel: w408 -> [w443]
                  i -> [w445]
                  stop <- w444 stop-if-true
                  n221 = Equal?(x=w443, y=w445) -> (x = y?=w444:bool)
                }
                n222 = while {
                  shift-right: [w433] -> _
                  shift-left: w399 -> [w439]
                  tunnel: w409 -> [w440]
                  tunnel: w398 -> [w437]
                  tunnel: w399 -> [w436]
                  tunnel: w401 -> [w432]
                  stop <- w435 continue-if-true
                  n223 = Increment(x=w439) -> (x+1=w441:u32)
                  n224 = Equal?(x=w439, y=w440) -> (x = y?=w434:bool)
                  n225 = xnode ("Memory Read")("Address"=w439) -> ("Data"=w438:i16)  [unwired: 1 in, 1 out]
                  n226 = Select(t=w436, s=w434, f=w441) -> (s? t:f=w433:u32)
                  n227 = Greater?(x=w432, y=w433) -> (0:→"End Linear Ramp":bool)
                  n228 = call "Loop Timer20"("Count(Ticks)"=w437) -> ()  [unwired: 1 out]
                  n229 = local read "Start Waveforms"() -> (w435:bool)
                  n230 = xnode "FPGA I/O Node"("Connector0/AO6"=w438) -> ()  [unwired: 1 in, 1 out]
                }
                n231 = node-c288(w406) -> ()
              }
              frame 7 {
                w459 = u16 0
                n232 = node-c288() -> (w464:T4)  [unwired: 1 in]
                n233 = while {
                  shift-right: [w512] -> _
                  shift-left: w465 -> [w518]
                  tunnel: w452 -> [w519]
                  tunnel: w453 -> [w516]
                  tunnel: w465 -> [w515]
                  stop <- w514 continue-if-true
                  n234 = Increment(x=w518) -> (x+1=w520:u32)
                  n235 = Equal?(x=w518, y=w519) -> (x = y?=w513:bool)
                  n236 = xnode ("Memory Read")("Address"=w518) -> ("Data"=w517:i16)  [unwired: 1 in, 1 out]
                  n237 = Select(t=w515, s=w513, f=w520) -> (s? t:f=w512:u32)
                  n238 = call "Loop Timer4"("Count(Ticks)"=w516) -> ()  [unwired: 1 out]
                  n239 = Less?(x=w512, y=u32 20) -> (x < y?=w510:bool)
                  n240 = xnode "FPGA I/O Node"("TRIG0"=w510) -> ()  [unwired: 1 in, 1 out]
                  n241 = local read "Start Waveforms"() -> (w514:bool)
                  n242 = xnode "FPGA I/O Node"("Connector0/AO1"=w517) -> ()  [unwired: 1 in, 1 out]
                }
                n243 = while {
                  shift-right: [w466] -> _
                  shift-left: FALSE -> [w489]
                  shift-right: [w483] -> _
                  shift-left: w459 -> [w485]
                  tunnel: w461 -> [w484]
                  shift-right: [w467] -> _
                  shift-left: w457 -> [w480]
                  tunnel: w460 -> [w479]
                  shift-right: [w473] -> _
                  shift-left: w459 -> [w476]
                  tunnel: w458 -> [w472]
                  tunnel: w457 -> [w469]
                  tunnel: w454 -> [w468]
                  stop <- w490 continue-if-true
                  n244 = local read "End Linear Ramp"() -> (w466:bool)
                  n245 = Increment(x=w485) -> (x+1=w488:u16)
                  n246 = Greater?(x=w466, y=w489) -> (0:w487:bool)
                  n247 = Select(t=w488, s=w487, f=w485) -> (s? t:f=w482:u16)
                  n248 = Add(x=w479, y=w480) -> (x+y=w481:i16)
                  n249 = Increment(x=w476) -> (x+1=w477:u16)
                  n250 = Equal?(x=w482, y=w484) -> (x = y?=w478:bool)
                  n251 = Select(t=u16 0, s=w478, f=w482) -> (s? t:f=w483:u16)
                  n252 = Select(t=w477, s=w478, f=w476) -> (s? t:f=w474:u16)
                  "frame counter" <- w474
                  n253 = Select(t=w481, s=w478, f=w480) -> (s? t:f=w475:i16)
                  n254 = call "Loop Timer17"("Count(Ticks)"=w468) -> ()  [unwired: 1 out]
                  n255 = Equal?(x=w474, y=w472) -> (x = y?=w471:bool)
                  n256 = local read "Start Waveforms"() -> (w490:bool)
                  n257 = Select(t=w469, s=w471, f=w475) -> (s? t:f=w467:i16)
                  n258 = xnode "FPGA I/O Node"("Connector0/AO3"=w467) -> ()  [unwired: 1 in, 1 out]
                  n259 = Select(t=u16 0, s=w471, f=w474) -> (s? t:f=w473:u16)
                }
                n260 = timed-loop {
                  timing: w464 -> [_]
                  timing-out: [_] -> w463
                  tunnel: w454 -> [w502]
                  tunnel: [w502] -> w455
                  tunnel: w451 -> [w503]
                  i -> [w505]
                  stop <- w504 stop-if-true
                  n261 = Equal?(x=w503, y=w505) -> (x = y?=w504:bool)
                }
                n262 = while {
                  shift-right: [w493] -> _
                  shift-left: w465 -> [w499]
                  tunnel: w450 -> [w500]
                  tunnel: w455 -> [w497]
                  tunnel: w465 -> [w496]
                  tunnel: w456 -> [w492]
                  stop <- w495 continue-if-true
                  n263 = Increment(x=w499) -> (x+1=w501:u32)
                  n264 = Equal?(x=w499, y=w500) -> (x = y?=w494:bool)
                  n265 = xnode ("Memory Read")("Address"=w499) -> ("Data"=w498:i16)  [unwired: 1 in, 1 out]
                  n266 = Select(t=w496, s=w494, f=w501) -> (s? t:f=w493:u32)
                  n267 = Greater?(x=w492, y=w493) -> (0:w491:bool)
                  n268 = local write "End Linear Ramp"(w491) -> ()
                  n269 = call "Loop Timer15"("Count(Ticks)"=w497) -> ()  [unwired: 1 out]
                  n270 = local read "Start Waveforms"() -> (w495:bool)
                  n271 = xnode "FPGA I/O Node"("Connector0/AO2"=w498) -> ()  [unwired: 1 in, 1 out]
                }
                n272 = node-c288(w463) -> ()
              }
            }
            n273 = case shown="4" w79 {
              frame 0, Default {
              }
              frame 3 {
                n274 = while {
                  stop <- w140 continue-if-true
                  n275 = local read "Start Waveforms"() -> (w140:bool)
                  n276 = xnode "FPGA I/O Node"("Connector0/AO1"="X Piezo Axis", "Connector0/AO2"="Y Piezo Axis", "Connector0/AO3"="Z Piezo Axis") -> ()  [unwired: 3 in, 3 out]
                }
              }
              frame 4 {
                n277 = local read "Galvo 1 Position (I16)"() -> (w142:i16)
                n278 = local read "Galvo 2 Position (I16)"() -> (w141:i16)
                n279 = xnode "FPGA I/O Node"("Connector0/AO5"=w142, "Connector0/AO6"=w141) -> ()  [unwired: 2 in, 2 out]
              }
            }
            n280 = Index Array(array="Accums Per Line", index #1=0 ("index"), index #2=1 ("index"), index #3=2 ("index"), index #4=3 ("index")) -> (element #1=w85:u32, element #2=w84:u32, element #3=w83:u32, element #4=w82:u32)
            n281 = Compound Arithmetic op=ADD(w85, w84, w83, w82) -> (w92:u32)
            n282 = Multiply(x="Number of Lines", y=w92) -> (x*y=w93:u32)
            n283 = node-c288() -> (w95:T4)  [unwired: 1 in]
            n284 = timed-loop {
              timing: w95 -> [_]
              timing-out: [_] -> w94
              shift-right: [w129] -> _
              shift-left: w81 -> [w109]
              shift-right: [w127] -> _
              shift-left: _ -> [w110]
              shift-right: [w128] -> _
              shift-left: _ -> [w126]
              shift-right: [w113] -> _
              shift-left: u32 0 -> [w118]
              shift-right: [w122] -> _
              shift-left: w81 -> [w120]
              tunnel: w93 -> [w117]
              tunnel: w79 -> [w111]
              stop <- "Stop Sync Signal" continue-if-true
              n285 = Increment(x=w118) -> (x+1=w121:u32)
              n286 = Equal?(x=w118, y=w117) -> (x = y?=w115:bool)
              n287 = And(x=w110, y=w120) -> (x .and. y?=w125:bool)
              n288 = And(x=w120, y=w110) -> (x .and. y?=w119:bool)
              n289 = local read "Frame Trigger"() -> (w124:bool)
              n290 = Select(t=w121, s=w119, f=w118) -> (s? t:f=w116:u32)
              n291 = case shown="True" w126 {
                tunnel: w125 -> [_ w132]
                frame False {
                }
                frame True {
                  n292 = xnode "FPGA I/O Node"("TRIG1"=w132) -> ()  [unwired: 1 in, 1 out]
                  "Laser Blank Trigger" <- w132
                }
              }
              n293 = xnode ("Register Write")("Data"=w109) -> ()  [unwired: 1 in, 1 out]
              n294 = case shown="5" w111 {
                tunnel: [w130 w131] -> w129
                frame 0, Default {
                  n295 = xnode "FPGA I/O Node"() -> ("Connector1/DIO0"=w130:bool)  [unwired: 1 in, 1 out]
                }
                frame 5 {
                  n296 = xnode ("Register Read")() -> ("Data"=w131:bool)  [unwired: 1 in, 1 out]
                }
              }
              n297 = Exclusive Or(1:w115, 2:w124) -> (0:w123:bool)
              n298 = Select(t=w124, s=w123, f=w120) -> (s? t:f=w122:bool)
              n299 = Select(t=u32 0, s=w115, f=w116) -> (s? t:f=w113:u32)
              n300 = Not Equal?(x=w129, y=w109) -> (x != y?=w128:bool)
              n301 = Greater?(x=w129, y=w109) -> (0:w127:bool)
            }
            n302 = node-c288(w94) -> ()
          }
        }
      }
    }
  }
  n303 = local read "Accums Per Line"() -> (w1:u32[])
  n304 = while {
    shift-right: [w564] -> _
    shift-left: u8 0 -> [w541]
    shift-right: [w565] -> _
    shift-left: w2 -> [w569]
    shift-right: [w563] -> _
    shift-left: u8 0 -> [w566]
    tunnel: "Sequences" -> [w562]
    shift-right: [w556] -> _
    shift-left: u32 0 -> [w557]
    tunnel: w1 -> [w543]
    shift-right: [w523] -> _
    shift-left: w2 -> [w538]
    stop <- FALSE stop-if-true
    n305 = local read "Laser Blank Trigger"() -> (w523:bool)
    n306 = To Long Integer(number=w541) -> (32bit integer=w540:i32)
    n307 = Add(x="Laser Delay (Ticks)", y="Laser On Time (Ticks)") -> (x+y=w527:u8)
    n308 = Index Array(array=w543, index=w540) -> (element=w542:u32)
    n309 = Increment(x=w557) -> (x+1=w558:u32)
    n310 = Equal?(x=w557, y=w542) -> (x = y?=w554:bool)
    n311 = Equal?(x=w566, y=w527) -> (x = y?=w555:bool)
    n312 = Greater?(x=w523, y=w538) -> (0:w537:bool)
    n313 = Select(t=w558, s=w555, f=w557) -> (s? t:f=w559:u32)
    n314 = Increment(x=w541) -> (x+1=w574:u8)
    n315 = Equal?(x=w541, y=w562) -> (x = y?=w571:bool)
    n316 = Exclusive Or(1:w555, 2:w537) -> (0:w570:bool)
    n317 = Select(t=u32 0, s=w554, f=w559) -> (s? t:f=w556:u32)
    n318 = Select(t=w574, s=w554, f=w541) -> (s? t:f=w573:u8)
    n319 = Increment(x=w566) -> (x+1=w568:u8)
    n320 = Select(t=w537, s=w570, f=w569) -> (s? t:f=w565:bool)
    n321 = Split Number(x="Laser States") -> (hi(x)=w551:u16, lo(x)=w552:u16)
    n322 = Select(t=u8 0, s=w571, f=w573) -> (s? t:f=w564:u8)
    n323 = Select(t=w568, s=w565, f=u8 0) -> (s? t:f=w563:u8)
    n324 = Split Number(x=w551) -> (hi(x)=w550:u8, lo(x)=w549:u8)
    n325 = Split Number(x=w552) -> (hi(x)=w548:u8, lo(x)=w547:u8)
    n326 = Greater?(x=w563, y="Laser Delay (Ticks)") -> (0:w539:bool)
    n327 = call "Loop Timer22"("Count(Ticks)"=u16 80) -> ()  [unwired: 1 out]
    n328 = case shown="0, Default" w564 {
      tunnel: w550 -> [w575 _ _ _]
      tunnel: w549 -> [_ w576 _ _]
      tunnel: w548 -> [_ _ w577 _]
      tunnel: w547 -> [_ _ _ w578]
      tunnel: [w575 w576 w577 w578] -> w546
      frame 0, Default {
      }
      frame 1 {
      }
      frame 2 {
      }
      frame 3 {
      }
    }
    n329 = Or(x="Blanking Off/Manual", y=w539) -> (x .or. y?=w522:bool)
    n330 = Select(t=w546, s=w522, f=u8 0) -> (s? t:f=w534:u8)
    n331 = Number To Boolean Array(number=w534) -> (Boolean array=w536:bool[])
    n332 = xnode "FPGA I/O Node"("Connector1/DIO4"="Blanking Off/Manual") -> ()  [unwired: 1 in, 1 out]
    n333 = Index Array(array=w536, index #1=0 ("index"), index #2=1 ("index"), index #3=2 ("index"), index #4=3 ("index")) -> (element #1=w530:bool, element #2=w529:bool, element #3=w525:bool, element #4=w524:bool)
    n334 = xnode "FPGA I/O Node"("Connector0/DIO0"=w530, "Connector1/DIO8"=w529, "Connector1/DIO9"=w525, "Connector1/DIO10"=w524) -> ()  [unwired: 4 in, 4 out]
  }
  n335 = while {
    stop <- "stop" stop-if-true
    n336 = call "Loop Timer23"("Count(uSec)"=u32 100) -> ()  [unwired: 1 out]
    n337 = xnode "FPGA I/O Node"("Connector1/DIO26"="Lower Shutter Command", "Connector1/DIO28"="Upper Shutter Command") -> ("Connector1/DIO25"=→"Lower Shutter Status":bool, "Connector1/DIO27"=→"Upper Shutter Status":bool)  [unwired: 4 in, 4 out]
  }
